vi "_lcod_CFX_ExecuteReguestAsync.vi"(8 "CFX_Message":refnum<vi>, 9 "timeout":dbl=15.0, 10 "Handle":string, 11 "ExecuteReouestAsync":refnum<k24>) -> (2 "CFX_Message_out":T1)   [LabVIEW 2025]
uses:
  CFX_dll/CFX.dll
panel:
  out "Elapsed Time (s)":dbl caption="已用时间(s)"
  out "error out":errorcluster caption="错误输出"
  in  "error in":errorcluster caption="错误输入"
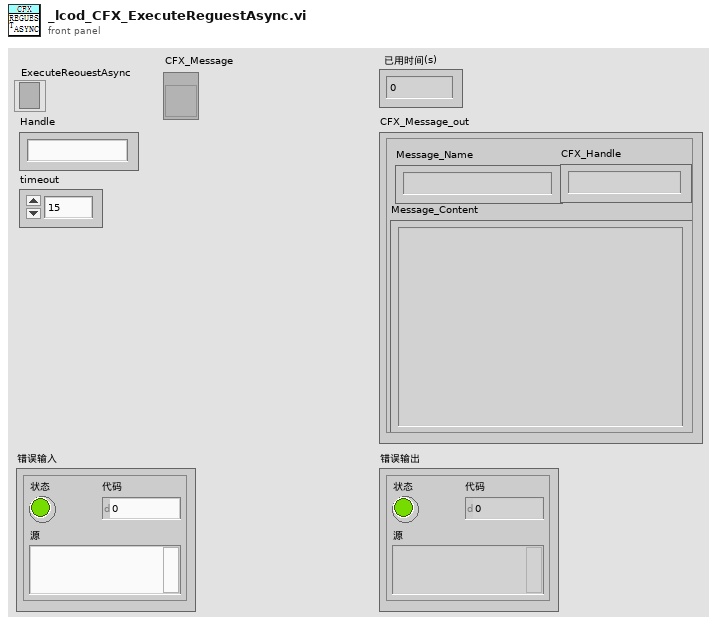
[diagram p1: front panel]
types:
  T1 = cluster{"Message_Name":string, "CFX_Handle":string, "Message_Content":string}
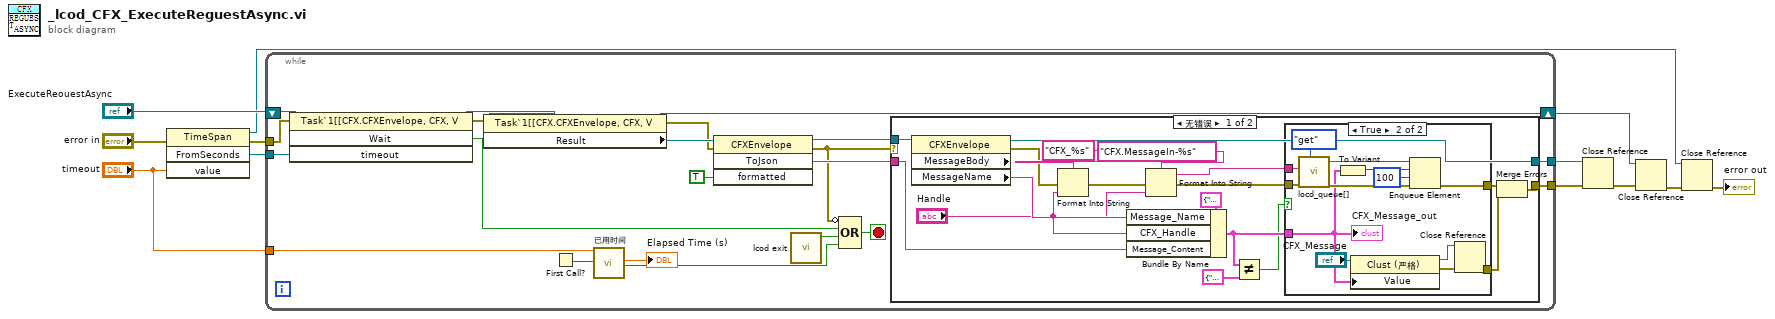
[diagram p0: block diagram]
diagram:
  n1 = invoke class="TimeSpan" method="FromSeconds"(error in="error in", "value"="timeout") -> (reference out=w1:refnum<k24>, error out=w10:errorcluster, "FromSeconds"=w9:refnum<k24>)  [unwired: 2 in, 1 out]
  n2 = while {
    tunnel: w10 -> [w32]
    tunnel: w9 -> [w31]
    shift-right: [w25] -> w4
    shift-left: "ExecuteReouestAsync" -> [w33]
    tunnel: "timeout" -> [w18]
    tunnel: [w14] -> w7
    tunnel: [w13] -> w6
    stop <- w27 stop-if-true
    n3 = invoke class="Task`1[[CFX.CFXEnvelope, CFX, V" method="Wait"(reference=w33, error in=w32, "timeout"=w31) -> (reference out=w30:refnum<k24>, error out=w29:errorcluster, "Wait"=w28:bool)  [unwired: 1 in, 1 out]
    n4 = property class="Task`1[[CFX.CFXEnvelope, CFX, V"(reference=w30, error in=w29) -> (reference out=w25:refnum<k24>, error out=w22:errorcluster, "Result"=w24:refnum<k24>)
    n5 = First Call?() -> (First Call?: T/F=w16:bool)
    n6 = call "已用时间"("Time Target (s)"=w18, "Reset"=w16) -> ("Elapsed Time (s)"=→"Elapsed Time (s)":dbl, "Time has Elapsed"=w17:bool)  [unwired: 10 in, 6 out]
    n7 = invoke on="调用节点" class="CFXEnvelope" method="ToJson"(reference=w24, error in=w22, "formatted"=TRUE) -> (reference out=w21:refnum<k24>, error out=w19:errorcluster, "ToJson"=w20:string)  [unwired: 1 in, 1 out]
    n8 = call "lcod exit.vi"() -> ("bExit out"=w26:bool)  [unwired: 11 in]
    n9 = Compound Arithmetic op=OR ("复合运算")(invert w19, w28, w26, w17) -> (w27:bool)
    n10 = case shown="无错误" w19 {
      selector: w19 -> [_ w67]
      tunnel: w21 -> [w51 w66]
      tunnel: w20 -> [w42 _]
      tunnel: [w39 w67] -> w14
      tunnel: [w37 w66] -> w13
      frame No Error {
        n11 = property class="CFXEnvelope" props=["MessageBody", "MessageName"](reference=w51) -> (reference out=w37:refnum<k24>, error out=w44:errorcluster, "MessageName"=w43:string)  [unwired: 1 in, 1 out]
        n12 = Format Into String(format string="CFX_%s" ("log_path"), error in=w44, "Handle") -> (error out=w50:errorcluster)  [unwired: 1 in, 1 out]
        n13 = Bundle By Name(cluster=T1 {"Message_Name"="", "CFX_Handle"="", "Message_Content"=""} ("CFX_Message_In"), "Message_Name"=w43, "CFX_Handle"="Handle", "Message_Content"=w42) -> (w36:T1)
        n14 = Format Into String(format string="CFX.MessageIn-%s" ("格式字符串"), error in=w50, "Handle") -> (resulting string=w48:string, error out=w49:errorcluster)  [unwired: 1 in]
        n15 = Not Equal?(x=w36, y=T1 {"Message_Name"="", "CFX_Handle"="", "Message_Content"=""} ("CFX_Message_out")) -> (x != y?=w34:bool)
        n16 = case shown="True" w34 {
          tunnel: w49 -> [w52 w64]
          tunnel: w48 -> [_ w61]
          tunnel: [w52 w58] -> w40
          tunnel: [_ w54] -> w38
          tunnel: w36 -> [_ w53]
          frame False {
          }
          frame True {
            n17 = call "locd_queue[].vi"("cmd"=enum16{"init", "get", "set", "end"}."get", "error in"=w64, "queue_name"=w61) -> ("error out"=w65:errorcluster, "queue_out"=w62:refnum<queue>)  [unwired: 4 in, 3 out]
            n18 = To Variant(anything=w53) -> (Variant=w63:variant)
            n19 = property class="Clust (严格)"(reference="CFX_Message", "Value"=w53) -> (reference out=w55:refnum<vi>, error out=w56:errorcluster)  [unwired: 1 in]
            n20 = Enqueue Element(queue=w62, element=w63, timeout in ms (-1)=100 ("超时毫秒(-1)"), error in (no error)=w65) -> (error out=w58:errorcluster)  [unwired: 2 out]
            n21 = Close Reference(reference=w55, error in (no error)=w56) -> (error out=w54:errorcluster)
            "CFX_Message_out" <- w53
          }
        }
        n22 = Merge Errors(w40, w38) -> (w39:errorcluster)
      }
      frame Error {
      }
    }
  }
  n23 = Close Reference(reference=w6, error in (no error)=w7) -> (error out=w5:errorcluster)
  n24 = Close Reference(reference=w4, error in (no error)=w5) -> (error out=w3:errorcluster)
  n25 = Close Reference(reference=w1, error in (no error)=w3) -> (error out=→"error out":errorcluster)
